vi "2D数组转1D数组.vi"(8 "列索引":i32, 9 "行索引":i32, 11 "2D表格":string[][](array[string])) -> (3 "1D表格":string[](array[string]))   [LabVIEW 2025]
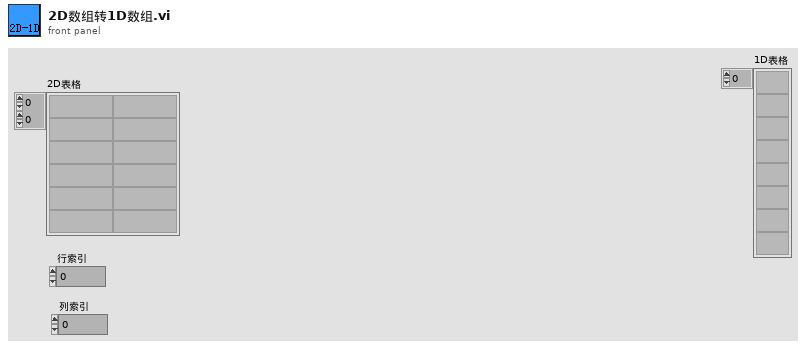
[diagram p1: front panel]
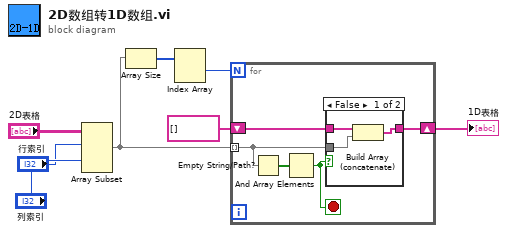
[diagram p0: block diagram]
diagram:
  n1 = Array Subset(array="2D表格", index (row)="行索引", index (col)="列索引") -> (w2:string[][])  [unwired: 2 in]
  n2 = Array Size(array=w2) -> (size(s)=w8:i32[])
  n3 = Index Array(array=w8) -> (element #1=w7:i32)  [unwired: 2 in, 1 out]
  n4 = for {
    N: w7 -> [_]
    tunnel: w2 -> [w11] mode=indexing
    shift-right: [w10] -> w5
    shift-left: string[] [] -> [w12]
    stop <- w9 stop-if-true
    n5 = Empty String/Path?(string/path=w11) -> (empty?=w13:bool[])
    n6 = And Array Elements(Boolean array=w13) -> (logical AND=w9:bool)
    n7 = case shown="False" w9 {
      tunnel: w12 -> [w16 w17]
      tunnel: w11 -> [w15 _]
      tunnel: [w14 w17] -> w10
      frame False {
        n8 = Build Array (concatenate)(w16, w15) -> (w14:string[])
      }
      frame True {
      }
    }
  }
  "1D表格" <- w5
